vi "Create Output Channels.vi"(8 "error in (no error)":errorcluster, 11 "Modbus in":refnum<class "Modbus.lvclass">) -> (0 "error out":errorcluster, 1 "Channels to remove":string[](array[string]), 3 "Modbus out":refnum<class "Modbus.lvclass">)   [LabVIEW 2026, in "Modbus.lvlib" / "Modbus.lvclass"]
uses:
  Modbus.lvclass
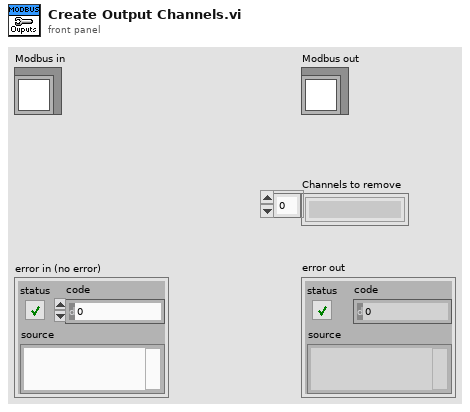
[diagram p1: front panel]
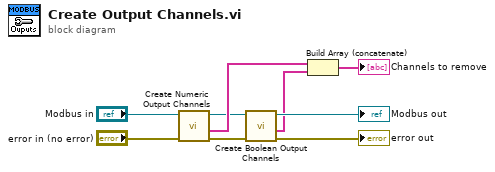
[diagram p0: block diagram]
diagram:
  n1 = call "Create Numeric Output Channels.vi"("error in (no error)"="error in (no error)", "Modbus in"="Modbus in") -> ("error out"=w2:errorcluster, "Channels to remove"=w4:string[], "Modbus out"=w3:refnum<class "Modbus.lvclass">)  [unwired: 7 in]
  n2 = call "Create Boolean Output Channels.vi"("error in (no error)"=w2, "Modbus in"=w3) -> ("error out"=→"error out":errorcluster, "Channels to remove"=w1:string[], "Modbus out"=→"Modbus out":refnum<class "Modbus.lvclass">)  [unwired: 7 in]
  n3 = Build Array (concatenate)(w4, w1) -> (→"Channels to remove":string[])
